vi "Read Monitor Channel.vi"(8 "error in":errorcluster, 10 "channel number in":u8, 11 "board handle in":u8) -> (0 "error out":errorcluster, 1 "monitor data out":T1[](array[typedef]), 2 "channel number out":u8, 3 "board handle out":u8)   [LabVIEW 2020, in "AIM ARINC 429 Hardware API.lvlib"]
uses:
  AIM ARINC 429 Hardware API.lvlib
  Monitor Data.ctl
  <instrlib>/AIM GmbH/_ARINC-429/AIM429LV.lvlib
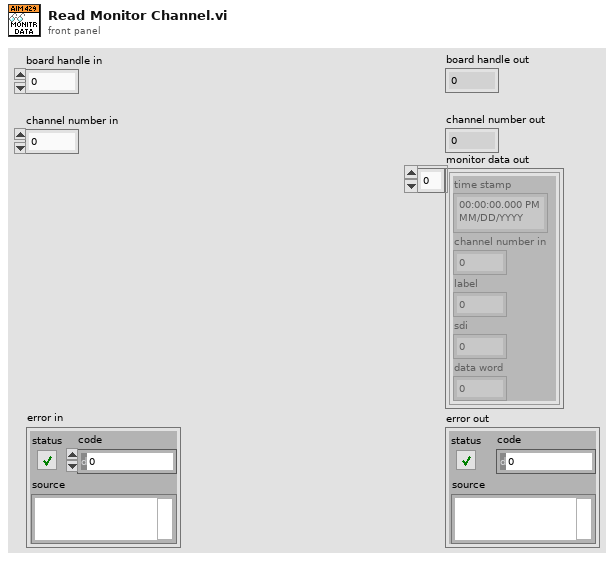
[diagram p1: front panel]
types:
  T1 = typedef "AIM ARINC 429 Hardware API.lvlib/Monitor Data.ctl" = cluster{"time stamp":timestamp, "channel number in":u8, "label":u8, "sdi":u8, "data word":u32}
  T2 = typedef "AIM429LV.lvlib/rx_stack_entry.ctl" = cluster{"label data":u32, "time tag":u32, "buffer report word":u32, "day of year":u32}
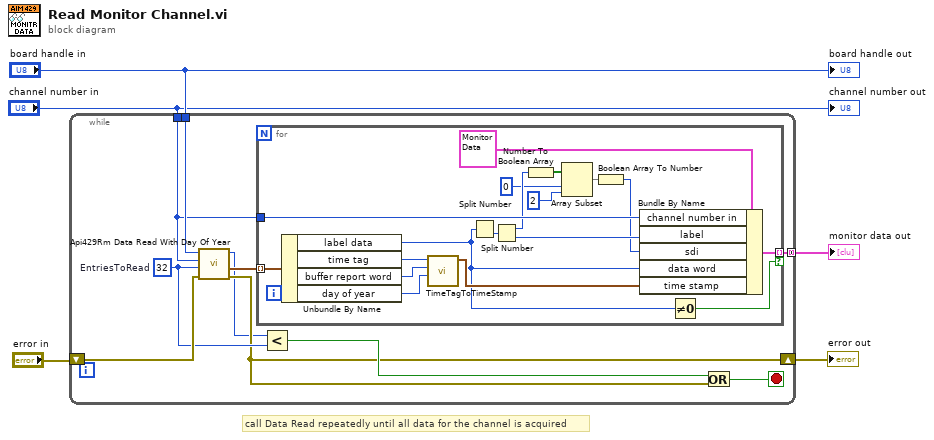
[diagram p0: block diagram]
diagram:
  # "call Data Read repeatedly until all data for the channel is acquired"
  n1 = while {
    tunnel: "board handle in" -> [w9]
    tunnel: "channel number in" -> [w7]
    shift-right: [w11] -> w2
    shift-left: "error in" -> [w13]
    tunnel: [w8] -> w1 mode=concatenating
    stop <- w14 stop-if-true
    w12 = u16 32  # EntriesToRead
    n2 = call <instrlib>:"Api429Rm Data Read With Day Of Year.vi"("error in"=w13, "uw_EntriesToRead"=w12, "b_Chn"=w7, "board_handle"=w9) -> ("error out"=w11:errorcluster, "px_SData"=w10:T2[], "puw_Count"=w6:u16)  [unwired: 5 in]
    n3 = for {
      tunnel: w10 -> [w33] mode=indexing
      tunnel: w7 -> [w28]
      tunnel: [w27] -> w8 mode=indexing if=w26
      n4 = Unbundle By Name(w33) -> ("label data"=w24:u32, "time tag"=w32:u32, "buffer report word"=w31:u32, "day of year"=w30:u32)
      n5 = call <instrlib>:"TimeTagToTimeStamp.vi"("day of year"=w30, "buffer report word"=w31, "time tag"=w32) -> ("time stamp"=w25:timestamp)  [unwired: 7 in, 1 out]
      n6 = Split Number(x=w24) -> (lo(x)=w23:u16)  [unwired: 1 out]
      n7 = Split Number(x=w23) -> (hi(x)=w21:u8, lo(x)=w22:u8)
      n8 = Number To Boolean Array(number=w21) -> (Boolean array=w20:bool[])
      n9 = Array Subset(array=w20, index=0, length=2) -> (w17:bool[])
      n10 = Boolean Array To Number(Boolean array=w17) -> (number=w16:u32)
      n11 = Bundle By Name(cluster=T1 {"time stamp"=timestamp(0 s since 1904-01-01), "channel number in"=0, "label"=0, "sdi"=0, "data word"=0} ("Word"), "channel number in"=w28, "label"=w22, "sdi"=w16, "data word"=w24, "time stamp"=w25) -> (w27:T1)
      n12 = Not Equal To 0?(x=w24) -> (x != 0?=w26:bool)
    }
    n13 = Less?(x=w6, y=w12) -> (x < y?=w15:bool)
    n14 = Or(x=w15, y=w11) -> (x .or. y?=w14:bool)
  }
  "error out" <- w2
  "monitor data out" <- w1
  "board handle out" <- "board handle in"
  "channel number out" <- "channel number in"
